vi "Barcode.vi"(11 "Barcode":string) -> (1 "Value ($)":dbl, 2 "Delay Time (s)":dbl, 3 "Actions":T1)   [LabVIEW 2026]
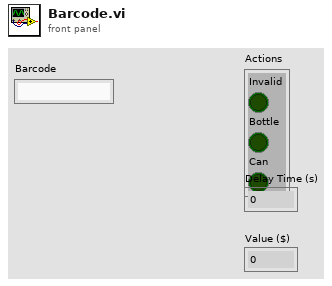
[diagram p1: front panel]
types:
  T1 = cluster{"Invalid":bool, "Bottle":bool, "Can":bool}
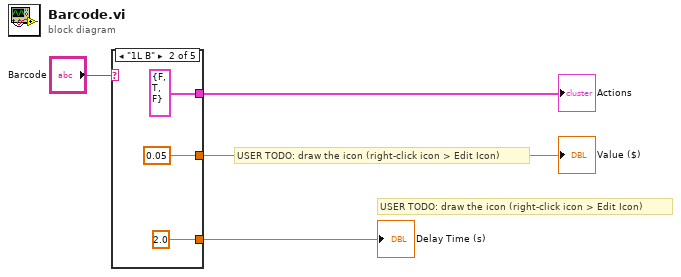
[diagram p0: block diagram]
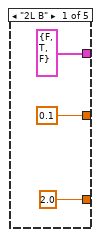
[diagram p2: hidden frame]
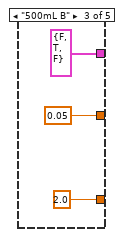
[diagram p3: hidden frame]
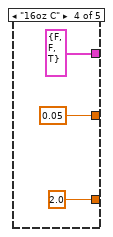
[diagram p4: hidden frame]
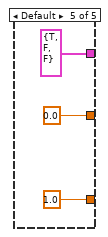
[diagram p5: hidden frame]
diagram:
  # "USER TODO: draw the icon (right-click icon > Edit Icon)"
  # "USER TODO: draw the icon (right-click icon > Edit Icon)"
  n1 = case shown="\"1L B\"" "Barcode" {
    tunnel: [T1 {"Invalid"=FALSE, "Bottle"=TRUE, "Can"=FALSE} ("Actions 2") T1 {"Invalid"=FALSE, "Bottle"=TRUE, "Can"=FALSE} ("Actions 2") T1 {"Invalid"=FALSE, "Bottle"=TRUE, "Can"=FALSE} ("Actions 2") T1 {"Invalid"=FALSE, "Bottle"=FALSE, "Can"=TRUE} ("Actions 2") T1 {"Invalid"=TRUE, "Bottle"=FALSE, "Can"=FALSE} ("Actions 2")] -> w3
    tunnel: [2.0 2.0 2.0 2.0 1.0] -> w2
    tunnel: [0.1 0.05 0.05 0.05 0.0] -> w1
    frame "2L B" {
    }
    frame "1L B" {
    }
    frame "500mL B" {
    }
    frame "16oz C" {
    }
    frame Default {
    }
  }
  "Actions" <- w3
  "Delay Time (s)" <- w2
  "Value ($)" <- w1
